vi "Init Events.vi"(8 "error in (no error)":errorcluster, 11 "SequenceViewPanel in":refnum<class "SequenceViewPanel.lvclass">) -> (0 "error out":errorcluster, 3 "SequenceViewPanel out":refnum<class "SequenceViewPanel.lvclass">)   [LabVIEW 2020, in "TSnax UI.lvlib" / "SequenceViewPanel.lvclass"]
uses:
  SequenceViewPanel.lvclass
  Set SequenceFile Request.ctl
  TSnax/SequenceFile/SequenceFile.lvclass
  Set SequenceFile Response.ctl
  Refresh Step Request.ctl
  TSnax/Step/Step.lvclass
  Error Response.ctl
  Mark Trace Data.ctl
  Trace Marker.ctl
  SequenceViewPanel.lvclass/SequenceViewPanel.ctl
  TSnax UI.lvlib
  Step Result Request.ctl
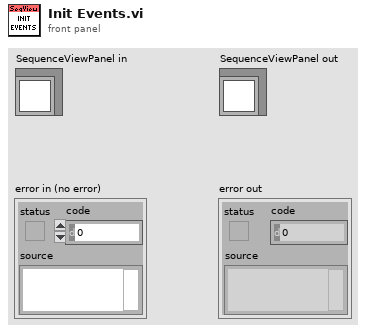
[diagram p1: front panel]
types:
  T1 = typedef "TSnax UI.lvlib/SequenceViewPanel.lvclass/Step Result Request.ctl" = cluster{"ID":string, "Result":string}
  T2 = typedef "TSnax UI.lvlib/SequenceViewPanel.lvclass/Mark Trace Data.ctl" = cluster{"Trace Marker":T3}
  T3 = typedef "TSnax UI.lvlib/SequenceViewPanel.lvclass/Trace Marker.ctl" = cluster{"TSnax:SequenceFile":refnum<class "SequenceFile.lvclass">, "SequenceIndex":i32, "StepGroup":i32, "PreviousStepIndex":i32, "NextStepIndex":i32}
  T4 = typedef "TSnax UI.lvlib/SequenceViewPanel.lvclass/Refresh Step Request.ctl" = cluster{"Step":refnum<class "Step.lvclass">, "Notifier":refnum<notifier>, "Auto-Release":bool}
  T5 = typedef "TSnax UI.lvlib/SequenceViewPanel.lvclass/Set SequenceFile Request.ctl" = cluster{"SequenceFile":refnum<class "SequenceFile.lvclass">, "Notifier":refnum<notifier>, "SequenceIndex":i32}
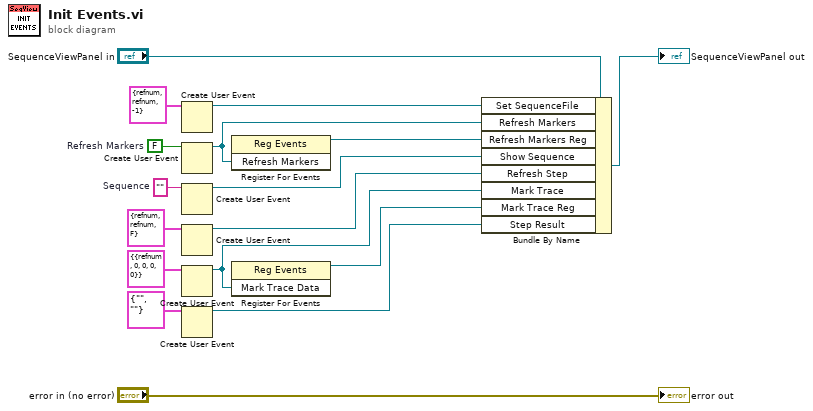
[diagram p0: block diagram]
diagram:
  w9 = ""  # Sequence
  w12 = FALSE  # Refresh Markers
  n1 = Create User Event(user event datatype=T5 {"SequenceFile"=refnum, "Notifier"=refnum, "SequenceIndex"=-1} ("Set SequenceFile")) -> (user event=w13:refnum<user-event>)  [unwired: 1 in, 1 out]
  n2 = Create User Event(user event datatype=w12) -> (user event=w11:refnum<user-event>)  [unwired: 1 in, 1 out]
  n3 = Create User Event(user event datatype=w9) -> (user event=w8:refnum<user-event>)  [unwired: 1 in, 1 out]
  n4 = Create User Event(user event datatype=T4 {"Step"=refnum, "Notifier"=refnum, "Auto-Release"=FALSE} ("Refresh Step Request")) -> (user event=w6:refnum<user-event>)  [unwired: 1 in, 1 out]
  n5 = Create User Event(user event datatype=T2 {"Trace Marker"={"TSnax:SequenceFile"=refnum, "SequenceIndex"=0, "StepGroup"=0, "PreviousStepIndex"=0, "NextStepIndex"=0}} ("Mark Trace Data")) -> (user event=w4:refnum<user-event>)  [unwired: 1 in, 1 out]
  n6 = Create User Event(user event datatype=T1 {"ID"="", "Result"=""} ("Step Result Request")) -> (user event=w1:refnum<user-event>)  [unwired: 1 in, 1 out]
  n7 = register-events(w11) -> (reference out=w10:refnum<event-registration>)  [unwired: 2 in, 1 out]
  n8 = register-events(w4) -> (reference out=w3:refnum<event-registration>)  [unwired: 2 in, 1 out]
  n9 = Bundle By Name(cluster="SequenceViewPanel in", "Set SequenceFile"=w13, "Refresh Markers"=w11, "Refresh Markers Reg"=w10, "Show Sequence"=w8, "Refresh Step"=w6, "Mark Trace"=w4, "Mark Trace Reg"=w3, "Step Result"=w1) -> (→"SequenceViewPanel out":refnum<class "SequenceViewPanel.lvclass">)
  "error out" <- "error in (no error)"
